vi "RFH-add-Permittivity_data.vi"() -> ()   [LabVIEW 2020, in "RFH-Reflection_File_Handler.lvlib"]
doc: "Run by hand: reads a common-format file, fills in the water or salt water model permittivity at the given water temperature (10-40 C) and saves it. The user picks the file."
uses:
  RFH-Reflection_File_Handler.lvlib
  RFH-common_data_format.ctl
  Computation/RDC-Reflection_Data_Computation.lvlib
panel:
  in  "water Temp (25C) [10-40C]":dbl=22.5 format="%#_13g"
  in  "file path perm source":path
  in  "file path (dialog if empty)":path
  out "Data":T1
  out "converted file path":path
  out "error out":errorcluster
  in  "error in (no error)":errorcluster
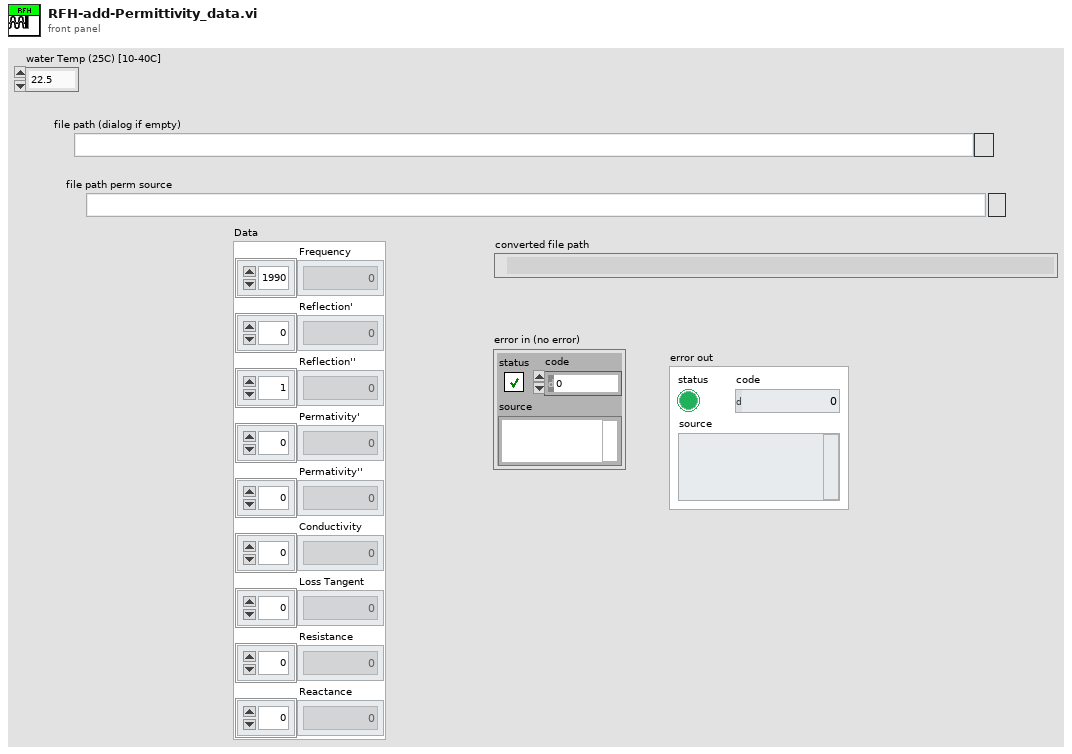
[diagram p1: front panel]
types:
  T1 = typedef "RFH-Reflection_File_Handler.lvlib/RFH-common_data_format.ctl" = cluster{"Frequency":dbl[], "Reflection'":dbl[], "Reflection''":dbl[], "Permativity'":dbl[], "Permativity''":dbl[], "Conductivity":dbl[], "Loss Tangent":dbl[], "Resistance":dbl[], "Reactance":dbl[]}
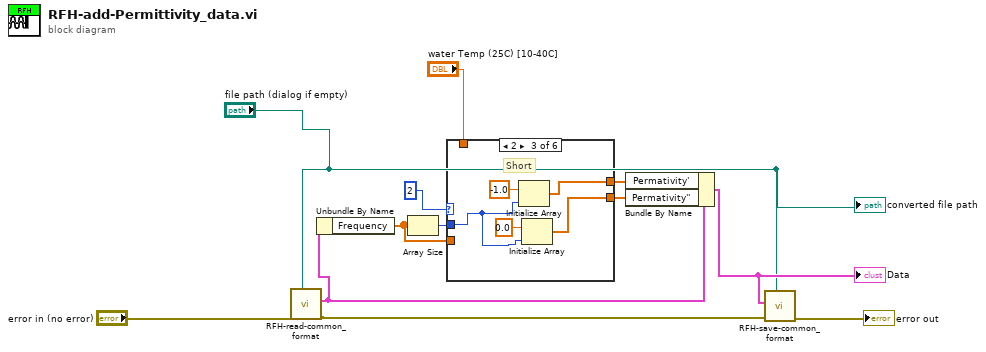
[diagram p0: block diagram]
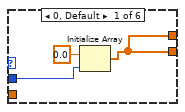
[diagram p2: hidden frame]
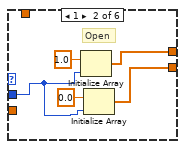
[diagram p3: hidden frame]
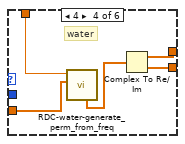
[diagram p4: hidden frame]
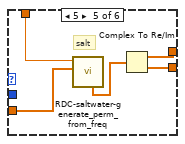
[diagram p5: hidden frame]
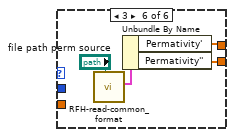
[diagram p6: hidden frame]
diagram:
  n1 = call "RFH-read-common_format.vi"("file path (dialog if empty)"="file path (dialog if empty)", "error in"="error in (no error)") -> ("error out"=w10:errorcluster, "Common Format"=w6:T1)  [unwired: 8 in]
  n2 = Unbundle By Name(w6) -> ("Frequency"=w2:dbl[])
  n3 = Array Size(array=w2) -> (size(s)=w3:i32)
  n4 = case shown="2" 2 {
    tunnel: [w13 w19 w24 w27 w34 w36] -> w7
    tunnel: [w13 w17 w22 w28 w35 w37] -> w5
    tunnel: w3 -> [w14 w16 w21 _ _ _]
    tunnel: w2 -> [_ _ _ w30 w33 _]
    tunnel: "water Temp (25C) [10-40C]" -> [_ _ _ w26 w31 _]
    frame 0, Default {
      n5 = Initialize Array(0.0 ("element"), w14) -> (w13:dbl[])
    }
    frame 1 {
      # "Open"
      n6 = Initialize Array(1.0 ("element"), w16) -> (w17:dbl[])
      n7 = Initialize Array(0.0 ("element"), w16) -> (w19:dbl[])
    }
    frame 2 {
      # "Short"
      n8 = Initialize Array(-1.0 ("element"), w21) -> (w22:dbl[])
      n9 = Initialize Array(0.0 ("element"), w21) -> (w24:dbl[])
    }
    frame 4 {
      # "water"
      n10 = call "RDC-water-generate_perm_from_freq.vi"("Frequency"=w30, "water Temp (25C) [10-40C]"=w26) -> ("Complex perm"=w29:cdb[])  [unwired: 5 in, 4 out]
      n11 = Complex To Re/Im(x + iy=w29) -> (x=w28:dbl[], y=w27:dbl[])
    }
    frame 5 {
      # "salt"
      n12 = call "RDC-saltwater-generate_perm_from_freq.vi"("Frequency"=w33, "water Temp (25C) [10-40C]"=w31) -> ("Complex perm"=w32:cdb[])  [unwired: 6 in, 3 out]
      n13 = Complex To Re/Im(x + iy=w32) -> (x=w35:dbl[], y=w34:dbl[])
    }
    frame 3 {
      n14 = call "RFH-read-common_format.vi"("file path (dialog if empty)"="file path perm source") -> ("Common Format"=w38:T1)  [unwired: 9 in, 1 out]
      n15 = Unbundle By Name(w38) -> ("Permativity'"=w37:dbl[], "Permativity''"=w36:dbl[])
    }
  }
  n16 = Bundle By Name(cluster=w6, "Permativity'"=w5, "Permativity''"=w7) -> (w9:T1)
  "Data" <- w9
  n17 = call "RFH-save-common_format.vi"("file path (use dialog)"="file path (dialog if empty)", "error in (no error)"=w10, "Common Format"=w9) -> ("error out"=→"error out":errorcluster)  [unwired: 8 in]
  "converted file path" <- "file path (dialog if empty)"
